vi "validate.vi"(8 "error in":errorcluster, 11 "EthernetIP configuration in":refnum<class "EIP Tags Configuration.lvclass">) -> (0 "error out":errorcluster, 3 "EthernetIP configuration out":refnum<class "EIP Tags Configuration.lvclass">)   [LabVIEW 2013, in "EIP Tags Configuration.lvclass"]
doc: "This function performs validation of the configuration. This function should be safe to call at any point and should not rely on anything in the runtime environment."
uses:
  EIP Tags Configuration.lvclass
  <vilib>/NI/Tag Bus Module Framework/module configuration/TBM module configuration.lvclass
  EIP Tags Configuration.lvclass/EIP Tags Configuration.ctl
  channel/EIP Tags Channel.lvclass/EIP Tags Channel.ctl
  channel/Read element.vi
  channel/Read EIP Tag UUID.vi
  channel/EIP Tags Channel.lvclass
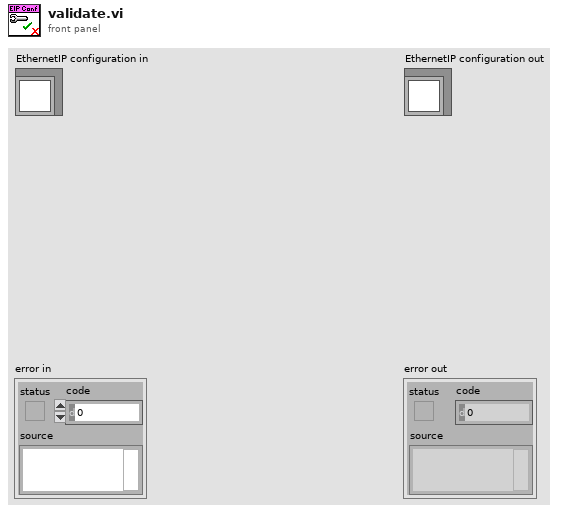
[diagram p1: front panel]
types:
  T1 = typedef "EIP Tags Configuration.lvclass/eip tag definition.ctl" = cluster{"eip tag types":T2, "unique tag name":string, "Number of Elements":u32}
  T2 = typedef "EIP Tags Configuration.lvclass/eip tag types.ctl" = enum16{"SINT", "INT", "DINT", "REAL", "BOOL", "STRING"}
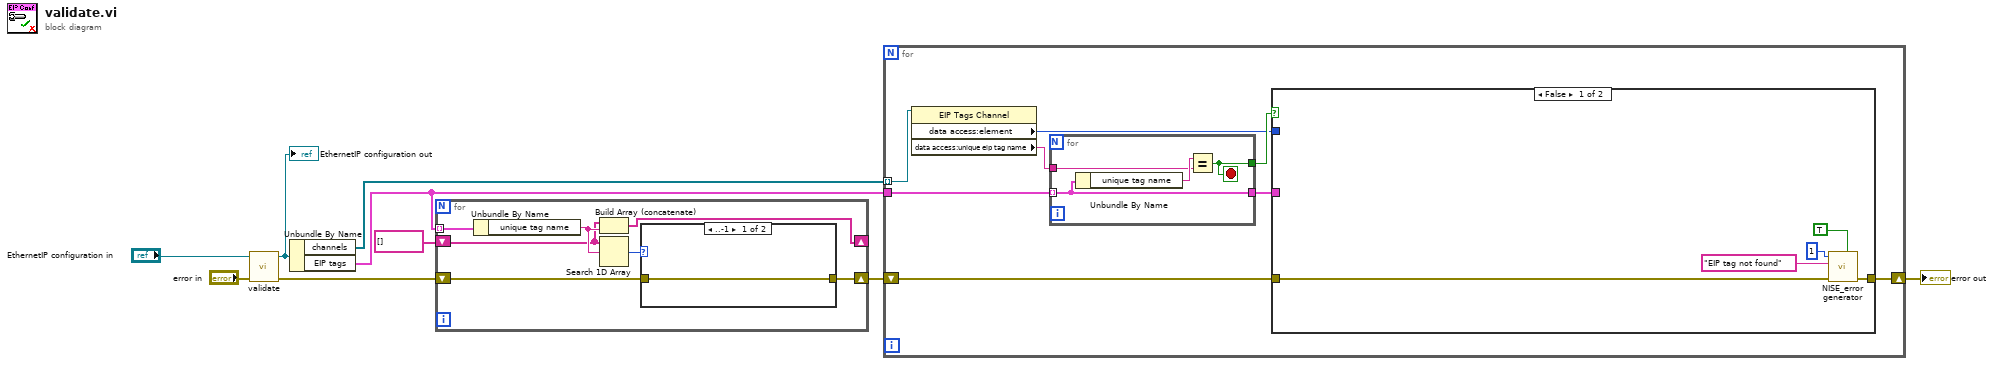
[diagram p0: block diagram]
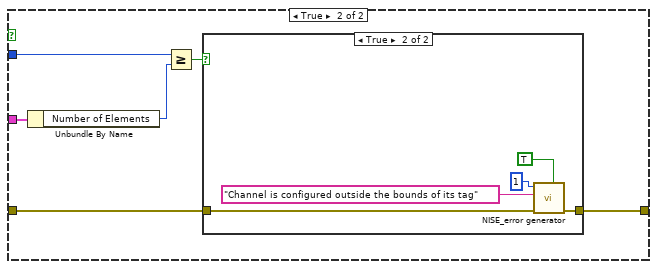
[diagram p2: hidden frame]
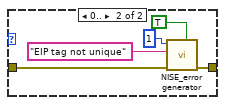
[diagram p4: hidden frame]
diagram:
  n1 = call-parent "validate.vi"("error in"="error in", "configuration in"="EthernetIP configuration in") -> ("error out"=w5:errorcluster, "configuration out"=w7:refnum<class "EIP Tags Configuration.lvclass">)  [unwired: 8 in]
  "EthernetIP configuration out" <- w7
  n2 = Unbundle By Name(w7) -> ("channels"=w4:refnum<class "EIP Tags Channel.lvclass">[], "EIP tags"=w3:T1[])
  n3 = for {
    tunnel: w3 -> [w16] mode=indexing
    shift-right: [w15] -> _
    shift-left: string[] [] -> [w13]
    shift-right: [w11] -> w2
    shift-left: w5 -> [w12]
    n4 = Unbundle By Name(w16) -> ("unique tag name"=w14:string)
    n5 = Build Array (concatenate)(w13, w14) -> (w15:string[])
    n6 = Search 1D Array(1D array=w13, element=w14) -> (index of element=w10:i32)  [unwired: 1 in]
    n7 = case shown="..-1" w10 {
      tunnel: w12 -> [w17 w21]
      tunnel: [w17 w22] -> w11
      frame ..-1 {
      }
      frame 0.. {
        n8 = call <vilib>:"NISE_error generator.vi"("concatenate (F)"=TRUE, "error in"=w21, "append error message"="EIP tag not unique" ("error message (\"\")"), "error code (0)"=1) -> ("error out"=w22:errorcluster)  [unwired: 5 in]
      }
    }
  }
  n9 = for {
    tunnel: w4 -> [w29] mode=indexing
    tunnel: w3 -> [w30]
    shift-right: [w24] -> w1
    shift-left: w2 -> [w25]
    n10 = property class="EIP Tags Channel"(reference=w29) -> ("data access:element"=w23:i32, "data access:unique eip tag name"=w28:string)  [unwired: 1 in, 2 out]
    n11 = for {
      tunnel: w30 -> [w49] mode=indexing
      tunnel: w28 -> [w50]
      tunnel: [w49] -> w26
      tunnel: [w48] -> w27
      stop <- w48 stop-if-true
      n12 = Unbundle By Name(w49) -> ("unique tag name"=w51:string)
      n13 = Equal?(x=w51, y=w50) -> (x = y?=w48:bool)
    }
    n14 = case shown="False" w27 {
      tunnel: w26 -> [_ w41]
      tunnel: w25 -> [w34 w37]
      tunnel: [w33 w38] -> w24
      tunnel: w23 -> [_ w36]
      frame False {
        n15 = call <vilib>:"NISE_error generator.vi"("concatenate (F)"=TRUE, "error in"=w34, "append error message"="EIP tag not found" ("error message (\"\")"), "error code (0)"=1) -> ("error out"=w33:errorcluster)  [unwired: 5 in]
      }
      frame True {
        n16 = Unbundle By Name(w41) -> ("Number of Elements"=w40:u32)
        n17 = Greater Or Equal?(x=w36, y=w40) -> (x >= y?=w39:bool)
        n18 = case shown="True" w39 {
          tunnel: [w42 w44] -> w38
          tunnel: w37 -> [w42 w45]
          frame False {
          }
          frame True {
            n19 = call <vilib>:"NISE_error generator.vi"("concatenate (F)"=TRUE, "error in"=w45, "append error message"="Channel is configured outside the bounds of its tag" ("error message (\"\")"), "error code (0)"=1) -> ("error out"=w44:errorcluster)  [unwired: 5 in]
          }
        }
      }
    }
  }
  "error out" <- w1
